vi "读设备返回值 - 步进电机 - MO1.vi"(8 "错误输入（无错误）":errorcluster, 9 "写/读":bool, 11 "VISA引用句柄输入":refnum<visa-resource-name>) -> (0 "错误输出":errorcluster, 1 "读取设备(n)":i32, 2 "报错":bool, 3 "VISA引用句柄输出":refnum<visa-resource-name>)   [LabVIEW 2026, in "UI-步进.lvlib"]
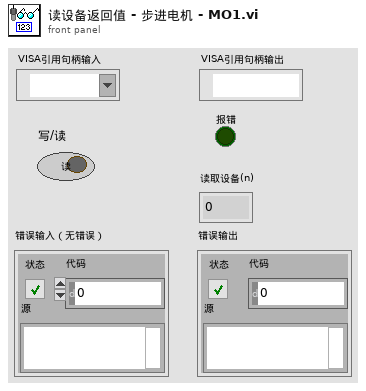
[diagram p1: front panel]
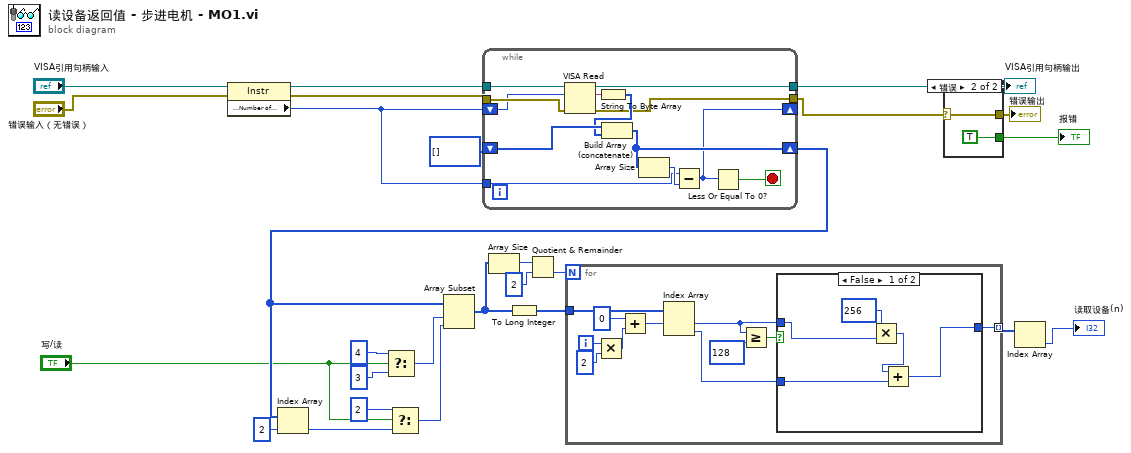
[diagram p0: block diagram]
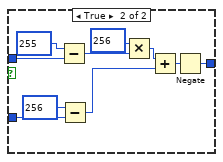
[diagram p2: hidden frame]
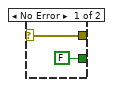
[diagram p3: hidden frame]
diagram:
  n1 = property class="Instr"(reference="VISA引用句柄输入", error in="错误输入（无错误）") -> (reference out=w23:refnum<visa-resource-name>, error out=w22:errorcluster, "Serial Settings:Number of Bytes at Serial Port"=w21:u32)
  n2 = Select(t=4 ("偏移量(0)"), s="写/读", f=3 ("偏移量(0)")) -> (s? t:f=w9:i32)
  n3 = while {
    tunnel: w23 -> [w37]
    tunnel: w22 -> [w36]
    shift-right: [w39] -> w6
    shift-left: u8[] [] ("unsigned byte array") -> [w38]
    tunnel: w21 -> [w31]
    shift-right: [w29] -> _
    shift-left: w21 -> [w35]
    tunnel: [w28] -> w20
    tunnel: [w27] -> w18
    stop <- w30 stop-if-true
    n4 = VISA Read(VISA resource name=w37, byte count=w35, error in (no error)=w36) -> (VISA resource name out=w28:refnum<visa-resource-name>, read buffer=w34:string, error out=w27:errorcluster)  [unwired: 1 out]
    n5 = String To Byte Array(string=w34) -> (unsigned byte array=w33:u8[])
    n6 = Build Array (concatenate)(w38, w33) -> (w39:u8[])
    n7 = Array Size(array=w39) -> (size(s)=w32:i32)
    n8 = Subtract(x=w31, y=w32) -> (x-y=w29:u32)
    n9 = Less Or Equal To 0?(x=w29) -> (x <= 0?=w30:bool)
  }
  "VISA引用句柄输出" <- w20
  n10 = Index Array(array=w6, index=2 ("索引")) -> (element=w1:u8)
  n11 = Select(t=2 ("偏移量(0)"), s="写/读", f=w1) -> (s? t:f=w8:i32)
  n12 = Array Subset(array=w6, index=w9, length=w8) -> (w7:u8[])
  n13 = Array Size(array=w7) -> (size(s)=w11:i32)
  n14 = To Long Integer(number=w7) -> (32bit integer=w13:i32[])
  n15 = Quotient & Remainder(x=w11, y=2) -> (floor(x/y)=w10:i32)  [unwired: 1 out]
  n16 = for {
    N: w10 -> [_]
    tunnel: w13 -> [w50]
    tunnel: [w41] -> w4 mode=indexing
    i -> [w48]
    n17 = Multiply(x=w48, y=2) -> (x*y=w46:i32)
    n18 = Add(x=0, y=w46) -> (x+y=w49:i32)
    n19 = Index Array(array=w50, index #1=w49) -> (element #1=w43:i32, element #2=w42:i32)  [unwired: 1 in]
    n20 = Greater Or Equal?(x=w43, y=128) -> (x >= y?=w45:bool)
    n21 = case shown="False" w45 {
      tunnel: w43 -> [w54 w63]
      tunnel: w42 -> [w52 w61]
      tunnel: [w51 w56] -> w41
      frame False {
        n22 = Multiply(x=256, y=w54) -> (x*y=w55:i32)
        n23 = Add(x=w55, y=w52) -> (x+y=w51:i32)
      }
      frame True {
        n24 = Subtract(x=255, y=w63) -> (x-y=w60:i32)
        n25 = Subtract(x=256, y=w61) -> (x-y=w58:i32)
        n26 = Multiply(x=256, y=w60) -> (x*y=w59:i32)
        n27 = Add(x=w59, y=w58) -> (x+y=w57:i32)
        n28 = Negate(x=w57) -> (-x=w56:i32)
      }
    }
  }
  n29 = case shown="错误" w18 {
    selector: w18 -> [w67 w68]
    tunnel: [w67 w68] -> w19
    tunnel: [FALSE TRUE] -> w17
    frame No Error {
    }
    frame Error {
    }
  }
  "错误输出" <- w19
  "报错" <- w17
  n30 = Index Array(array=w4) -> (element=→"读取设备(n)":i32)  [unwired: 1 in]
